vi "Init.vi"(8 "error in (no error)":errorcluster, 11 "DAQNavi_AI in":refnum<class "DAQNavi_AI.lvclass">) -> (0 "error out":errorcluster, 3 "DAQNavi_AI out":refnum<class "DAQNavi_AI.lvclass">)   [LabVIEW 2021, in "DAQNavi_AI.lvclass"]
uses:
  DAQNavi_AI.lvclass
  DAQNavi_AI.lvclass/DAQNavi_AI.ctl
  <userlib>/DAQNavi Polymorphic VI/create/DAQNavi Create Channel(AI-Voltage).vi
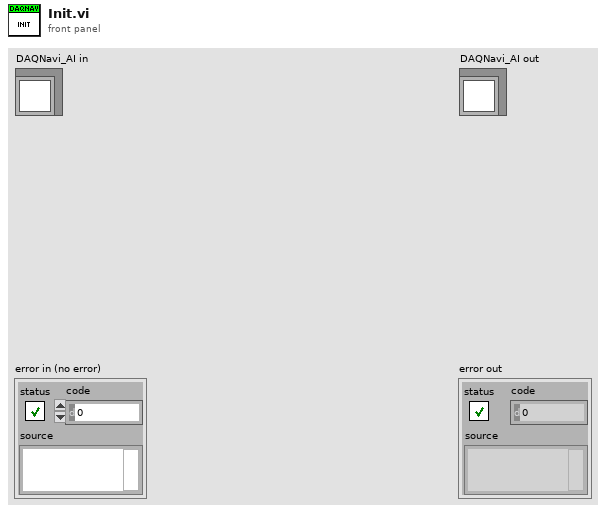
[diagram p1: front panel]
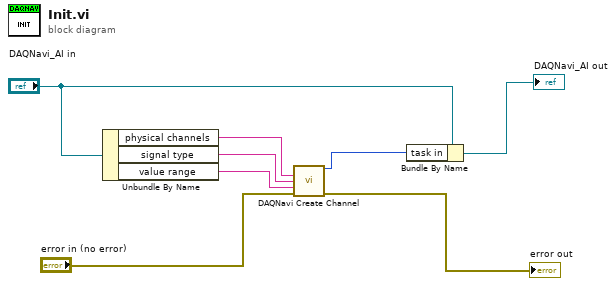
[diagram p0: block diagram]
diagram:
  n1 = Unbundle By Name("DAQNavi_AI in") -> ("physical channels"=w7:string, "signal type"=w6:string, "value range"=w5:string)
  n2 = call-poly <userlib>:"DAQNavi Create Channel.vi"("physical channels"=w7, "signal type"=w6, "value range"=w5, "error in (no error)"="error in (no error)") -> ("task out"=w2:i32, "error out"=→"error out":errorcluster)  [unwired: 10 in]
  n3 = Bundle By Name(cluster="DAQNavi_AI in", "task in"=w2) -> (→"DAQNavi_AI out":refnum<class "DAQNavi_AI.lvclass">)
